vi "VeriStand FPGA Generation Wizard.vi"() -> ()   [LabVIEW 2025]
uses:
  Classes/Project/Project.lvclass
panel:
  in  "Peeping?":bool
  in  "WebBrowser":refnum<k7>(container)
  in  "Export":bool
  in  "error in":errorcluster
  in  "Exit":bool
  in  "Build":bool
  in  "IO CSV Path":path
  in  "Project Path":path
  out "error out":errorcluster
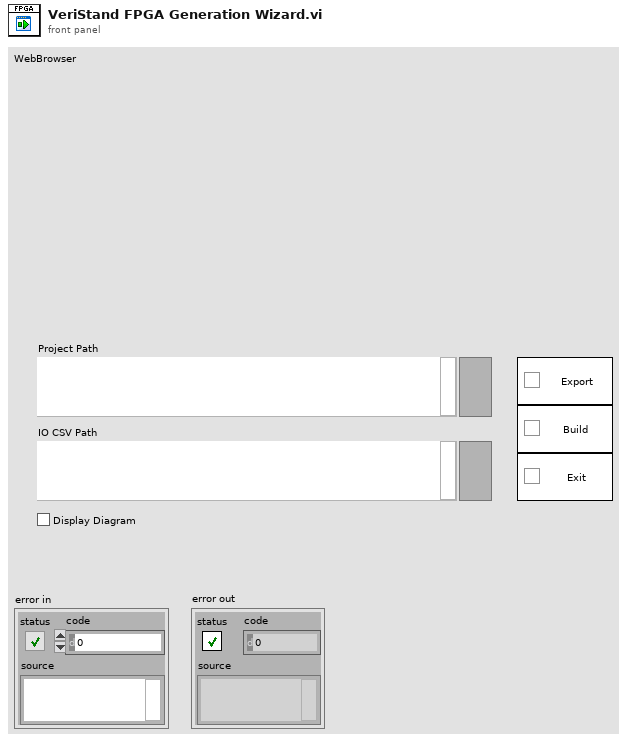
[diagram p1: front panel]
types:
  T1 = typedef "Project.lvclass/FPGA Settings.ctl" = cluster{"FPGA Target Name":string, "Modules":T2[]}
  T2 = typedef "Module.lvclass/Module Settings.ctl" = cluster{"Group Name":string, "Model Number":string, "Signals":T3[]}
  T3 = typedef "Signal.lvclass/Signal Settings.ctl" = cluster{"Signal Name":string, "IO Name":string, "Signal Type":string, "Signal Parameters":string, "IO Resource":string}
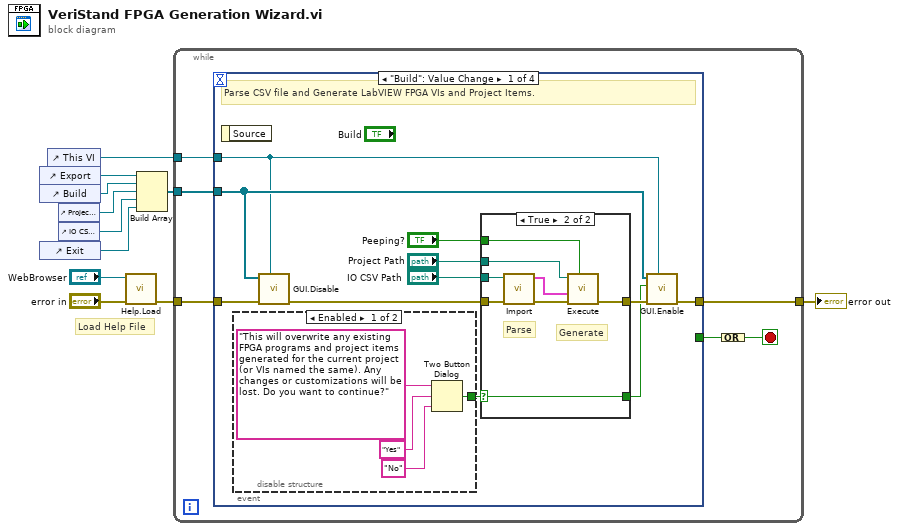
[diagram p0: block diagram]
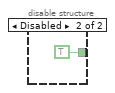
[diagram p2: hidden frame]
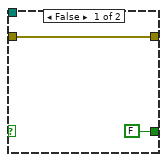
[diagram p3: hidden frame]
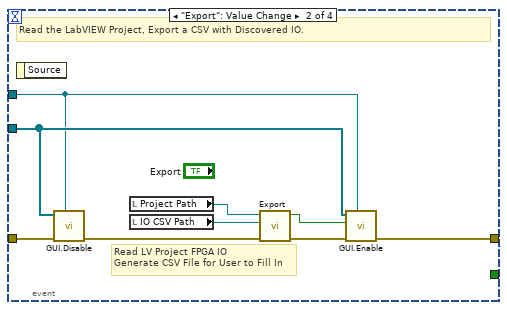
[diagram p4: hidden frame]
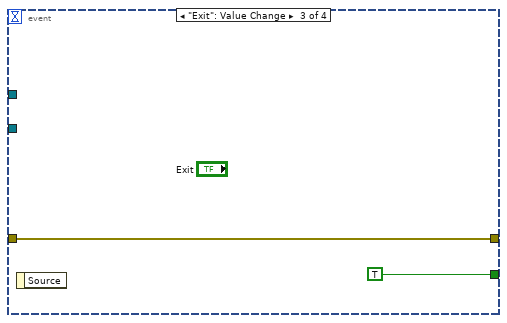
[diagram p5: hidden frame]
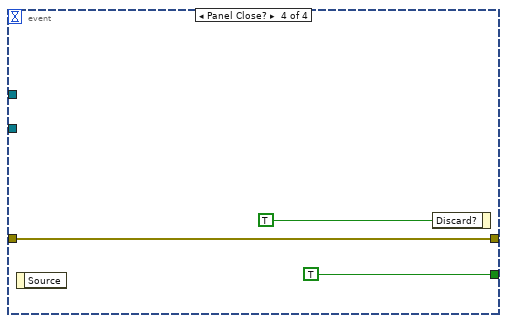
[diagram p6: hidden frame]
diagram:
  # "Load Help File"
  n1 = control-ref of="Export"() -> (w1:refnum<vi>)
  n2 = control-ref of="Build"() -> (w10:refnum<vi>)
  n3 = control-ref of="Exit"() -> (w7:refnum<vi>)
  n4 = control-ref of="This VI"() -> (w2:refnum<vi>)
  n5 = control-ref of="Project Path"() -> (w9:refnum<vi>)
  n6 = control-ref of="IO CSV Path"() -> (w8:refnum<vi>)
  n7 = call "Help.Load.vi"("error in (no error)"="error in", "Web Browser Reference"="WebBrowser") -> ("error out"=w4:errorcluster)  [unwired: 9 in]
  n8 = Build Array(w1, w10, w9, w8, w7) -> (w6:refnum<vi>[])
  n9 = while {
    tunnel: w6 -> [w14]
    tunnel: w2 -> [w13]
    tunnel: w4 -> [w17]
    tunnel: [w12] -> w11
    stop <- w15 stop-if-true
    n10 = event shown="[0] \"Build\": Value Change" {
      selector: _ -> [_ _ _ _]
      dyn-events: _ -> [_ _ _ _]
      timeout: _ -> [_ _ _ _]
      tunnel: [w22 w50 w54 w57] -> w12
      tunnel: w17 -> [w23 w51 w54 w57]
      tunnel: [_ _ TRUE TRUE] -> w16
      tunnel: w14 -> [w24 w52 _ _]
      tunnel: w13 -> [w21 w45 _ _]
      event "Build": Value Change {
        # "Parse CSV file and Generate LabVIEW FPGA VIs and Project Items."
        n11 = event-data() -> ()  [unwired: 1 in, 1 out]
        n12 = disable-structure shown="Enabled" {
          disable-tunnel: [w29 TRUE ("T button?")] -> w20
          frame Enabled {
            n13 = Two Button Dialog(message="This will overwrite any existing FPGA programs and project items generated for the current project (or VIs named the same). Any changes or customizations will be lost. Do you want to continue?", 1:"No" ("F button name (\"Cancel\")"), 2:"Yes" ("T button name (\"OK\")")) -> (T button?=w29:bool)
          }
          frame Disabled {
          }
        }
        n14 = call "GUI.Disable.vi"("VI reference (current VI)"=w21, "error in (no error)"=w23, "Array"=w24) -> ("error out"=w26:errorcluster)  [unwired: 8 in]
        n15 = case shown="True" w20 {
          selector: w20 -> [_ w37]
          tunnel: "Project Path" -> [_ w43]
          tunnel: "IO CSV Path" -> [_ w40]
          tunnel: w26 -> [w35 w39]
          tunnel: [w35 w38] -> w25
          tunnel: [FALSE w37] -> w19
          tunnel: "Peeping?" -> [_ w36]
          frame False {
          }
          frame True {
            # "Generate"
            # "Parse"
            n16 = call "Import.vi"("error in"=w39, "CSV Path"=w40) -> ("error out"=w42:errorcluster, "FPGA Settings"=w41:T1[])  [unwired: 8 in]
            n17 = call "Execute.vi"("Peeping?"=w36, "error in (no error)"=w42, "Targets"=w41, "Project Path"=w43) -> ("error out"=w38:errorcluster)  [unwired: 7 in]
          }
        }
        n18 = call "GUI.Enable.vi"("VI reference (current VI)"=w21, "error in (no error)"=w25, "Ran?"=w19, "Array"=w24) -> ("error out"=w22:errorcluster)  [unwired: 7 in]
      }
      event "Export": Value Change {
        # "Read LV Project FPGA IO\nGenerate CSV File for User to Fill In"
        # "Read the LabVIEW Project, Export a CSV with Discovered IO."
        n19 = event-data() -> ()  [unwired: 1 in, 1 out]
        n20 = call "GUI.Disable.vi"("VI reference (current VI)"=w45, "error in (no error)"=w51, "Array"=w52) -> ("error out"=w47:errorcluster)  [unwired: 8 in]
        n21 = local read "Project Path"() -> (w49:path)
        n22 = local read "IO CSV Path"() -> (w48:path)
        n23 = call "Export.vi"("error in (no error)"=w47, "Export Path"=w48, "Project Path"=w49) -> ("error out"=w46:errorcluster, "Ran?"=w44:bool)  [unwired: 7 in]
        n24 = call "GUI.Enable.vi"("VI reference (current VI)"=w45, "error in (no error)"=w46, "Ran?"=w44, "Array"=w52) -> ("error out"=w50:errorcluster)  [unwired: 7 in]
      }
      event "Exit": Value Change {
        n25 = event-data() -> ()  [unwired: 1 in, 1 out]
      }
      event Panel Close? {
        n26 = event-data() -> ()  [unwired: 1 in, 1 out]
        n27 = event-data("Discard?"=TRUE) -> ()  [unwired: 1 in, 1 out]
      }
    }
    n28 = Compound Arithmetic op=OR(w16) -> (w15:bool)
  }
  "error out" <- w11
